vi "ModernNetworkStreamer.vi"   [LabVIEW 2026]
uses:
  StateMachine/Globals.vi
types:
  T1 = typedef "IMAQ Image.ctl" = refnum<image>
  T2 = typedef "System_State.ctl" = u16
  T3 = cluster{"ClrCount 1":i32, "ClrCount 2":i32, "ClrCount 3":i32, "ClrCount 4":i32, "Throughput (obj/min)":dbl, "ClrGate 1":bool, "ClrGate 2":bool, "ClrGate 3":bool, "ClrGate 4":bool, "Data String":string, "System State":T2}
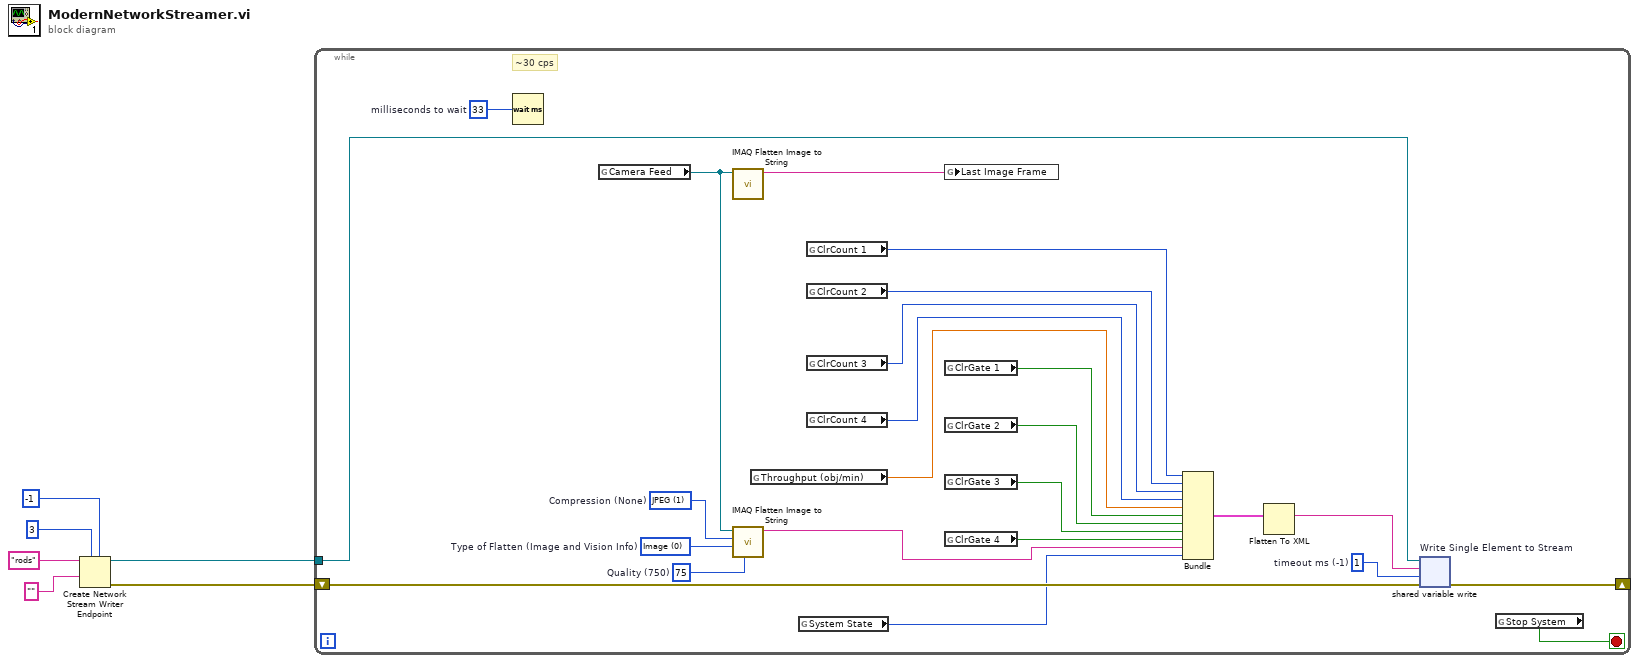
[diagram p0: block diagram]
diagram:
  n1 = Create Network Stream Writer Endpoint(5:-1 ("timeout in ms (-1)"), 7:3 ("writer buffer size"), 9:"" ("writer name"), 11:"rods" ("writer name")) -> (0:w1:errorcluster, 3:w3:refnum<k21>)  [unwired: 3 in]
  n2 = while {
    tunnel: w3 -> [w19]
    shift-right: [w11] -> _
    shift-left: w1 -> [w12]
    stop <- w29 stop-if-true
    w13 = 75  # Quality (750)
    w14 = 0 items=["Image", "Image and Vision Info", "Reference to Image"]  # Type of Flatten (Image and Vision Info)
    w15 = 1 items=["None", "JPEG", "PACKED BINARY"]  # Compression (None)
    w16 = 1  # timeout ms (-1)
    w30 = u32 33  # milliseconds to wait
    # "~30 cps"
    n3 = Wait (ms)(milliseconds to wait=w30) -> ()  [unwired: 1 out]
    n4 = global read "Globals.vi" "Camera Feed"() -> (w8:T1)
    n5 = call "IMAQ Flatten Image to String"("Image"=w8) -> ("Data String"=w7:string)  [unwired: 9 in, 1 out]
    n6 = call "IMAQ Flatten Image to String"("Quality (750)"=w13, "Type of Flatten (Image and Vision Info)"=w14, "Compression (None)"=w15, "Image"=w8) -> ("Data String"=w9:string)  [unwired: 6 in, 1 out]
    n7 = global read "Globals.vi" "Throughput (obj/min)"() -> (w24:dbl)
    n8 = global read "Globals.vi" "System State"() -> (w10:T2)
    n9 = global read "Globals.vi" "ClrCount 1"() -> (w28:i32)
    n10 = global read "Globals.vi" "ClrCount 2"() -> (w27:i32)
    n11 = global read "Globals.vi" "ClrCount 3"() -> (w26:i32)
    n12 = global read "Globals.vi" "ClrCount 4"() -> (w25:i32)
    n13 = global write "Globals.vi" "Last Image Frame"(w7) -> ()
    n14 = global read "Globals.vi" "ClrGate 1"() -> (w23:bool)
    n15 = global read "Globals.vi" "ClrGate 2"() -> (w22:bool)
    n16 = global read "Globals.vi" "ClrGate 3"() -> (w21:bool)
    n17 = global read "Globals.vi" "ClrGate 4"() -> (w20:bool)
    n18 = Bundle "Bundle"("ClrCount 1"=w28, "ClrCount 2"=w27, "ClrCount 3"=w26, "ClrCount 4"=w25, "Throughput (obj/min)"=w24, "ClrGate 1"=w23, "ClrGate 2"=w22, "ClrGate 3"=w21, "ClrGate 4"=w20, "Data String"=w9, "System State"=w10) -> (w18:T3)  [unwired: 1 in]
    n19 = Flatten To XML(6:w18) -> (2:w17:string)
    n20 = shared-variable-write "Write Single Element to Stream"(w19, w12, w17, w16) -> (w11:errorcluster)  [unwired: 2 out]
    n21 = global read "Globals.vi" "Stop System"() -> (w29:bool)
  }
